vi "Core Read U8 FIFO.vi"(7 "Include Header":bool, 8 "error in (no error)":errorcluster, 9 "Timeout (ms)":i32, 11 "CIFFIFO in":refnum<class "CIF_CIPC_Fifo_U8.lvclass">) -> (0 "error out":errorcluster, 1 "timed out?":bool, 3 "CIFFIFO out":refnum<class "CIF_CIPC_Fifo_U8.lvclass">)   [LabVIEW 2021, in "CIF_CIPC_Fifo_U8.lvclass"]
uses:
  CIF_CIPC_Fifo_U8.lvclass
  C:/Program Files/National Instruments/LabVIEW 2021/vi.lib/CIF Foundation/CIF Channels Core/CIFChannels/CIFChannels.lvclass
  D:/dev/Packages/CIF_Channels_CIPC/src/CIPC_Channels/CIF_CIPC_Chan/CIF_CIPC_Chn.lvclass
  <vilib>/CIF Foundation/CIF Channels Core/ChannelCommon/typedef/Channel State.ctl
  <vilib>/CIF Foundation/CIF Channels Core/ChannelCommon/typedef/Direction.ctl
  <vilib>/CIF Foundation/CIF Channels Core/CIFChannels/CIFChannels.lvclass/CIFChannels.ctl
  <vilib>/CIF Foundation/CIF CIPC/TypeDefs/Data Element Details.ctl
  <vilib>/CIF Foundation/CIF CIPC/TypeDefs/Read Configuration.ctl
  <vilib>/CIF Foundation/CIF CIPC/TypeDefs/Read Position.ctl
  CIF_CIPC_Chan/CIF_CIPC_Chn.lvclass/CIF_CIPC_Chn.ctl
  CIF_CIPC_Fifo_U8.lvclass/CIF_CIPC_Fifo_U8.ctl
  <vilib>/CIF Foundation/CIF Utilities/Statistics/I64/Stats_I64_CIF_U.lvclass/Stats_I64_CIF_U.ctl
  e703c505-0034-46a9-8989-21c0de27793f.vi
  768488f4-e6df-4560-a449-a64b33b49031.vi
  <vilib>/CIF Foundation/CIF Channels Core/CIFChannels/Accessors/Read Channel State.vi
  <vilib>/CIF Foundation/CIF Channels Core/CIFChannels/Accessors/Read Direction.vi
  <vilib>/CIF Foundation/CIF Utilities/DataTypes/Flatten Unflatten/Unflatten U64.vi
  <vilib>/CIF Foundation/CIF Utilities/DataTypes/Flatten Unflatten/Unflatten I64.vi
  <vilib>/CIF Foundation/CIF Channels Core/ChannelCommon/Utilities/Add Error.vi
  CIF_CIPC_Chan/Accessors/Read CIPC Channel.vi
  Read Wrapper for Backpressure Support.vi/b5615cf0-cd7f-4476-b9a9-d6ef7628cc3b.vi
  CIF_CIPC_Chan/Accessors/Read Buffer Configuration.vi
  Read Wrapper for Backpressure Support.vi/6248fc70-cc83-4025-b778-a3221b95feac.vi
  <vilib>/CIF Foundation/CIF Channels Core/CIFChannels/Accessors/Read FIFO Backpressure.vi
  <vilib>/CIF Foundation/CIF Utilities/Statistics/I64/X1 minus X0.vi
  <vilib>/CIF Foundation/CIF Utilities/Time/System Time/Get System Time.vi
  <vilib>/CIF Foundation/CIF CIPC/SubVIs/Wait For N Elements Available.vi
  <vilib>/CIF Foundation/CIF CIPC/SubVIs/Get Element Read Position.vi
  <vilib>/CIF Foundation/CIF CIPC/SubVIs/Check Error.vi
  <vilib>/CIF Foundation/CIF CIPC/SubVIs/Get dll Path.vi
  <vilib>/CIF Foundation/CIF CIPC/SubVIs/Set Element Read Position.vi
  Read Wrapper for Backpressure Support.vi/6248fc70-cc83-4025-b778-a3221b95feac.vi/331f6ecb-7ec4-4931-b93d-4fbd8d66a851.vi
  Read Wrapper for Backpressure Support.vi/6248fc70-cc83-4025-b778-a3221b95feac.vi/5ce0d4cf-f921-42ba-b14c-c90f7f7611e4.vi
  <vilib>/CIF Foundation/CIF Utilities/Statistics/I64/X1 minus X0.vi/dfabcf33-0dbc-4041-80a5-3dc0c86d2989.vi
  <vilib>/CIF Foundation/CIF CIPC/SubVIs/Notify Of New Write.vi
  <vilib>/CIF Foundation/CIF CIPC/SubVIs/Get Element Write Position.vi
  <vilib>/CIF Foundation/CIF Utilities/Statistics/I64/X1 minus X0.vi/dfabcf33-0dbc-4041-80a5-3dc0c86d2989.vi/9eb60a9a-770f-4d2d-8b3f-8465c267ecc9.vi
  <vilib>/CIF Foundation/CIF CIPC/SubVIs/Check Error Core.vi
  <vilib>/CIF Foundation/CIF CIPC/SubVIs/Get Element Info Variant.vi
  <vilib>/CIF Foundation/CIF Channels Core/ChannelCommon/Utilities/Add Error Core.vi
  <vilib>/CIF Foundation/CIF Channels Core/ChannelCommon/ChannelCommon.lvlib
  <vilib>/CIF Foundation/CIF Channels Core/CIFChannels/CIFChannels.lvclass
  <vilib>/CIF Foundation/CIF CIPC/CIF_NI_CIPC.lvlib
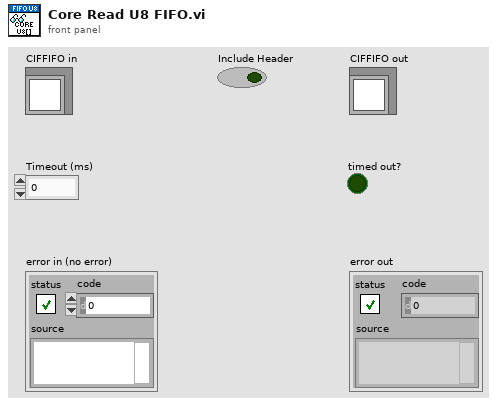
[diagram p1: front panel]
types:
  T1 = typedef "ChannelCommon.lvlib/Channel State.ctl" = enum8{"Creating", "Disconnected", "Connecting", "Connected", "Destroyed"}
  T2 = typedef "ChannelCommon.lvlib/Direction.ctl" = enum8{"Publisher", "Subscriber"}
  T3 = typedef "CIF_NI_CIPC.lvlib/Data Element Details.ctl" = cluster{"Bytes to Read":u32, "Element Offset":u32}
  T4 = typedef "CIF_NI_CIPC.lvlib/Read Configuration.ctl" = cluster{"Read Position":T5, "Element Offset":i32, "Prepend Array Size":bool, "Get Read Position":bool}
  T5 = typedef "CIF_NI_CIPC.lvlib/Read Position.ctl" = enum8{"Next", "Newest", "Oldest", "Next Available", "Absolute"}
  T6 = typedef "ChannelCommon.lvlib/FIFO Header.ctl" = cluster{"Length":u64, "T0":i64, "T_Out":i64, "T_Tx":i64, "Ctr":u64, "ClockID":u8}
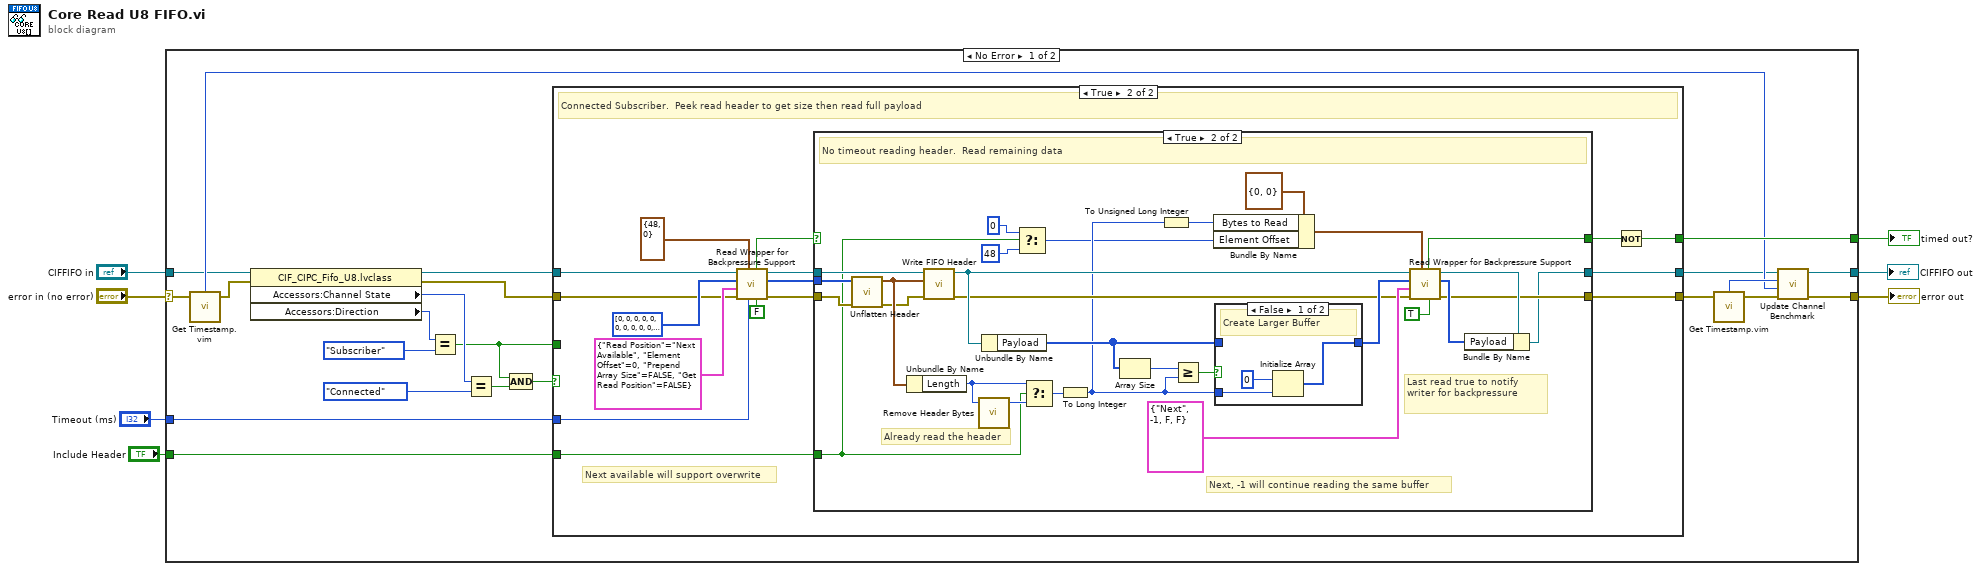
[diagram p0: block diagram]
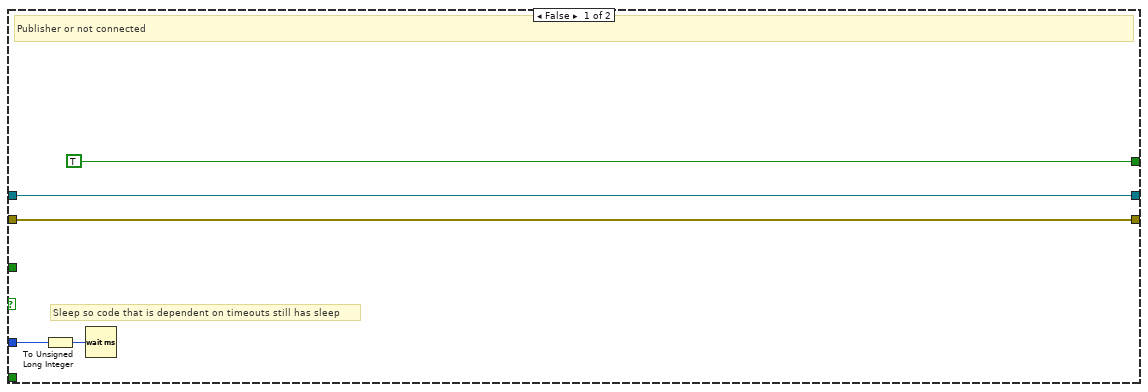
[diagram p2: hidden frame]
diagram:
  n1 = case shown="No Error" "error in (no error)" {
    selector: "error in (no error)" -> [w11 w88]
    tunnel: [w17 w88] -> w2
    tunnel: [w18 w87] -> w3
    tunnel: "CIFFIFO in" -> [w10 w87]
    tunnel: [w29 _] -> w4
    tunnel: "Timeout (ms)" -> [w19 _]
    tunnel: "Include Header" -> [w8 _]
    frame No Error {
      n2 = call "Get Timestamp.vim"("Anything in"=w11) -> ("Time (ns)"=w15:i64, "Anything out"=w9:errorcluster)  [unwired: 2 in]
      n3 = property class="CIF_CIPC_Fifo_U8.lvclass"(reference=w10, error in=w9) -> (reference out=w28:refnum<class "CIF_CIPC_Fifo_U8.lvclass">, error out=w27:errorcluster, "Accessors:Channel State"=w24:T1, "Accessors:Direction"=w26:T2)
      n4 = Equal?(x=w26, y=Direction."Subscriber") -> (x = y?=w20:bool)
      n5 = Equal?(x=w24, y=Channel_State."Connected") -> (x = y?=w22:bool)
      n6 = Compound Arithmetic op=AND(w20, w22) -> (w21:bool)
      n7 = case shown="True" w21 {
        tunnel: [TRUE ("timeout out") w47] -> w29
        tunnel: w27 -> [w33 w38]
        tunnel: w28 -> [w34 w37]
        tunnel: w20 -> [_ _]
        tunnel: [w34 w50] -> w13
        tunnel: [w33 w49] -> w12
        tunnel: w19 -> [w31 w41]
        tunnel: w8 -> [_ w35]
        frame False {
          # "Sleep so code that is dependent on timeouts still has sleep"
          # "Publisher or not connected"
          n8 = To Unsigned Long Integer(number=w31) -> (unsigned 32bit integer=w30:u32)
          n9 = Wait (ms)(milliseconds to wait=w30) -> ()  [unwired: 1 out]
        }
        frame True {
          # "Next available will support overwrite"
          # "Connected Subscriber.  Peek read header to get size then read full payload"
          n10 = call "Read Wrapper for Backpressure Support.vi"("Last Read"=FALSE, "Timeout (ms)"=w41, "Data Element"=T3 {"Bytes to Read"=48, "Element Offset"=0}, "error in (no error)"=w38, "Read Configuration"=T4 {"Read Position"=enum."Next Available", "Element Offset"=0, "Prepend Array Size"=FALSE, "Get Read Position"=FALSE}, "Data in"=u8[] [0, 0, 0, 0, 0, 0, 0, 0, 0, 0, 0, 0, 0, 0, 0, 0, 0, 0, 0, 0, 0, 0, 0, 0, 0, 0, 0, 0, 0, 0, 0, 0, 0, 0, 0, 0, 0, 0, 0, 0, 0, 0, 0, 0, 0, 0, 0, 0] ("U8 Array in"), "CIF_CIPC_Fifo_U8 in"=w37) -> ("error out"=w40:errorcluster, "Data out"=w39:u8[], "CIF_CIPC_Fifo_U8 out"=w46:refnum<class "CIF_CIPC_Fifo_U8.lvclass">, "Success"=w44:bool)  [unwired: 1 out]
          n11 = case shown="True" w44 {
            selector: w44 -> [w51 _]
            tunnel: w46 -> [w53 w70]
            tunnel: w40 -> [w52 w82]
            tunnel: w39 -> [_ w81]
            tunnel: [w52 w66] -> w49
            tunnel: [w53 w65] -> w50
            tunnel: [w51 w63] -> w48
            tunnel: w35 -> [_ w57]
            frame False {
              # "Timeout reading header"
            }
            frame True {
              # "Last read true to notify writer for backpressure"
              # "Already read the header"
              # "Next, -1 will continue reading the same buffer"
              # "No timeout reading header.  Read remaining data"
              n12 = call <vilib>:"Unflatten Header.vi"("error in (no error)"=w82, "Flattened Data in"=w81) -> ("error out"=w68:errorcluster, "Header out"=w69:T6)  [unwired: 7 in, 1 out]
              n13 = Unbundle By Name(w69) -> ("Length"=w60:u64)
              n14 = call <vilib>:"Write FIFO Header.vi"("error in (no error)"=w68, "Header"=w69, "CIFChannels in"=w70) -> ("error out"=w64:errorcluster, "CIFChannels out"=w67:refnum<class "CIF_CIPC_Fifo_U8.lvclass">)  [unwired: 7 in]
              n15 = call <vilib>:"Remove Header Bytes.vi"("Bytes/Msg with header"=w60) -> ("Bytes/Msg without header"=w59:u64)  [unwired: 3 in]
              n16 = Unbundle By Name(w67) -> ("Payload"=w78:u8[])
              n17 = Select(t=u32 0 ("Element Offset"), s=w57, f=u32 48 ("Element Offset")) -> (s? t:f=w54:u32)
              n18 = Select(t=w60, s=w57, f=w59) -> (s? t:f=w58:u64)
              n19 = To Long Integer(number=w58) -> (32bit integer=w62:i32)
              n20 = Array Size(array=w78) -> (size(s)=w79:i32)
              n21 = To Unsigned Long Integer(number=w62) -> (unsigned 32bit integer=w77:u32)
              n22 = Greater Or Equal?(x=w79, y=w62) -> (x >= y?=w80:bool)
              n23 = Bundle By Name(cluster=T3 {"Bytes to Read"=0, "Element Offset"=0} ("Data Element"), "Bytes to Read"=w77, "Element Offset"=w54) -> (w71:T3)
              n24 = case shown="False" w80 {
                tunnel: w78 -> [_ w86]
                tunnel: [w85 w86] -> w75
                tunnel: w62 -> [w83 _]
                frame False {
                  # "Create Larger Buffer"
                  n25 = Initialize Array(u8 0, w83) -> (w85:u8[])
                }
                frame True {
                  # "Reuse buffer"
                }
              }
              n26 = call "Read Wrapper for Backpressure Support.vi"("Last Read"=TRUE, "Data Element"=w71, "error in (no error)"=w64, "Read Configuration"=T4 {"Read Position"=enum."Next", "Element Offset"=-1, "Prepend Array Size"=FALSE, "Get Read Position"=FALSE}, "Data in"=w75, "CIF_CIPC_Fifo_U8 in"=w67) -> ("error out"=w66:errorcluster, "Data out"=w73:u8[], "CIF_CIPC_Fifo_U8 out"=w72:refnum<class "CIF_CIPC_Fifo_U8.lvclass">, "Success"=w63:bool)  [unwired: 1 in, 1 out]
              n27 = Bundle By Name(cluster=w72, "Payload"=w73) -> (w65:refnum<class "CIF_CIPC_Fifo_U8.lvclass">)
            }
          }
          n28 = Not(x=w48) -> (.not. x?=w47:bool)
        }
      }
      n29 = call "Get Timestamp.vim"("Anything in"=w12) -> ("Time (ns)"=w16:i64, "Anything out"=w14:errorcluster)  [unwired: 2 in]
      n30 = call <vilib>:"Update Channel Benchmark.vi"("error in (no error)"=w14, "X0"=w15, "X1"=w16, "CIFChannels in"=w13) -> ("error out"=w17:errorcluster, "CIFChannels out"=w18:refnum<class "CIF_CIPC_Fifo_U8.lvclass">)  [unwired: 6 in]
    }
    frame Error {
    }
  }
  "error out" <- w2
  "timed out?" <- w4
  "CIFFIFO out" <- w3
